vi "Actor Core.vi"(8 "error in":errorcluster, 11 "ZM-ROOT-root in":refnum<class "ZM-ROOT-root.lvclass">) -> (0 "error out":errorcluster, 3 "Actor out":refnum<class "Actor.lvclass">)   [LabVIEW 2020, in "ZM-ROOT-root.lvlib" / "ZM-ROOT-root.lvclass"]
doc: "Actor Core override of the root. ZM-ROOT-init launches the CM and the HWM and registers for the panel events before Call Parent; ZM-ROOT-helperPanel runs beside Call Parent. After Call Parent, ZM-ROOT-stop ends the panel loop and ZM-ROOT-close destroys the events. Error-handling plan: none yet; an error stops the root, and AF's Stop Core stops the children."
uses:
  ZM-ROOT-root.lvclass
  <vilib>/ActorFramework/Actor/Actor.lvclass
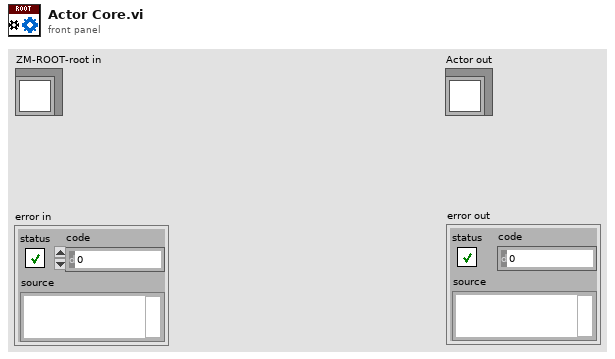
[diagram p1: front panel]
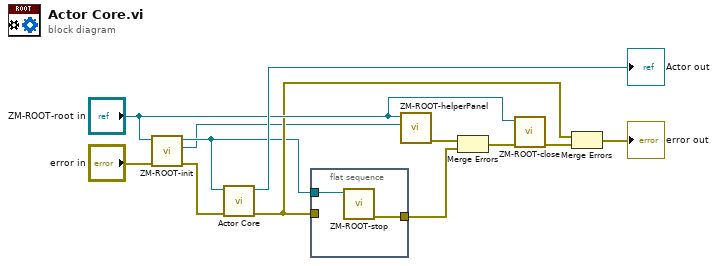
[diagram p0: block diagram]
diagram:
  n1 = call "ZM-ROOT-init.vi"("error in"="error in", "ZM-ROOT-root in"="ZM-ROOT-root in") -> ("error out"=w2:errorcluster, "event registration refnum"=w1:refnum<event-registration>, "ZM-ROOT-root out"=w3:refnum<class "ZM-ROOT-root.lvclass">)  [unwired: 7 in]
  n2 = call-parent "Actor Core.vi"("error in"=w2, "Actor in"=w3) -> ("error out"=w6:errorcluster, "Actor out"=→"Actor out":refnum<class "Actor.lvclass">)  [unwired: 8 in]
  n3 = flat-sequence {
    tunnel: w3 -> [w14]
    tunnel: [w13] -> w7
    tunnel: w6 -> [_]
    frame #0 {
      n4 = call "ZM-ROOT-stop.vi"("ZM-ROOT-root in"=w14) -> ("error out"=w13:errorcluster)  [unwired: 9 in, 1 out]
    }
  }
  n5 = call "ZM-ROOT-helperPanel.vi"("event registration refnum"=w1, "ZM-ROOT-root in"="ZM-ROOT-root in") -> ("error out"=w9:errorcluster)  [unwired: 9 in]
  n6 = Merge Errors(w9, w7) -> (w8:errorcluster)
  n7 = call "ZM-ROOT-close.vi"("error in (no error)"=w8, "ZM-ROOT-root in"="ZM-ROOT-root in") -> ("error out"=w5:errorcluster)  [unwired: 8 in, 1 out]
  n8 = Merge Errors(w6, w5) -> (→"error out":errorcluster)
